vi "Create MCP SSE Response.vi"(8 "error in (no error)":errorcluster) -> (0 "error out":errorcluster, 1 "cancelled":refnum<queue>, 2 "events":refnum<queue>, 3 "MCP SSE Response out":refnum<class "MCP SSE Response.lvclass">)   [LabVIEW 2020, in "MCP Server.lvlib" / "MCP SSE Response.lvclass"]
doc: "Creates an MCP SSE Response ready to be returned from an IG HTTP Server request handler. Obtains the events queue (string; one complete, formatted SSE event per element, an empty string ends the stream) and the cancelled flag (a single-element Boolean queue, initialised to FALSE and set to TRUE by Abort Stream), stores both in the object, and sets status 200 and the headers Content-Type: text/event-stream, Cache-Control: no-cache, X-Accel-Buffering: no and Transfer-Encoding: chunked. The IG HTTP Server frames a response of unknown length in chunks but does not add that header itself; without it a client reads the chunk sizes as part of the body. The caller owns both queues and must release them when the stream is finished."
uses:
  MCP SSE Response.lvclass
  C:/Program Files/National Instruments/LabVIEW 2026/vi.lib/IlluminatedG/IG HTTP Utils/HTTP Utils/Response/Response.lvclass
  MCP SSE Response.lvclass/MCP SSE Response.ctl
  <vilib>/IlluminatedG/IG HTTP Utils/HTTP Utils/Response/Response.lvclass
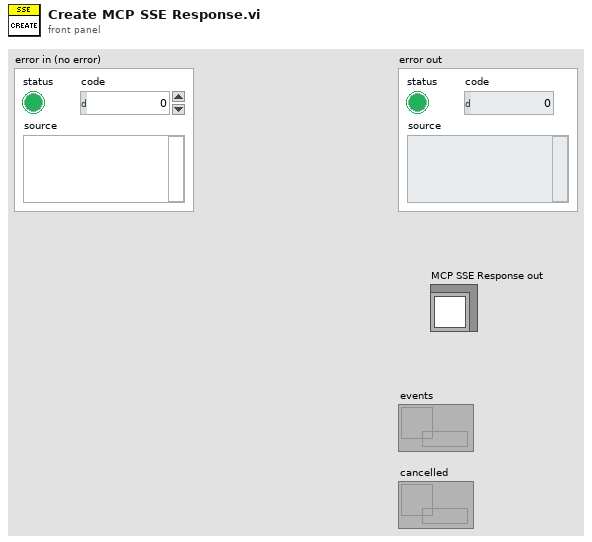
[diagram p1: front panel]
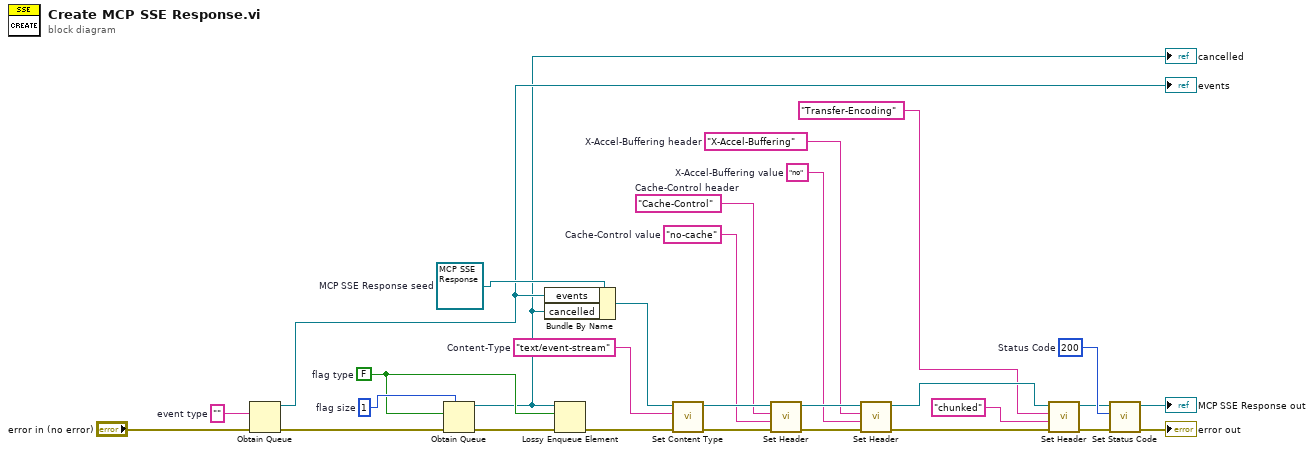
[diagram p0: block diagram]
diagram:
  w11 = u16 200  # Status Code
  w12 = "no"  # X-Accel-Buffering value
  w13 = "X-Accel-Buffering"  # X-Accel-Buffering header
  w16 = "no-cache"  # Cache-Control value
  w17 = "Cache-Control"  # Cache-Control header
  w20 = "text/event-stream"  # Content-Type
  w26 = 1  # flag size
  w25 = FALSE  # flag type
  w29 = ""  # event type
  w23 = refnum<class "MCP SSE Response.lvclass"> refnum  # MCP SSE Response seed
  n1 = Obtain Queue(element data type=w29, error in (no error)="error in (no error)") -> (queue out=w8:refnum<queue>, error out=w27:errorcluster)  [unwired: 3 in, 1 out]
  "events" <- w8
  n2 = Obtain Queue(max queue size (-1, unlimited)=w26, element data type=w25, error in (no error)=w27) -> (queue out=w7:refnum<queue>, error out=w24:errorcluster)  [unwired: 2 in, 1 out]
  "cancelled" <- w7
  n3 = Bundle By Name(cluster=w23, "events"=w8, "cancelled"=w7) -> (w21:refnum<class "MCP SSE Response.lvclass">)
  n4 = Lossy Enqueue Element(queue=w7, element=w25, error in (no error)=w24) -> (error out=w22:errorcluster)  [unwired: 3 out]
  n5 = call <vilib>:"Set Content Type.vi"("error in (no error)"=w22, "Content-Type"=w20, "Response in"=w21) -> ("error out"=w19:errorcluster, "Response out"=w18:refnum<class "MCP SSE Response.lvclass">)  [unwired: 7 in]
  n6 = call <vilib>:"Set Header.vi"("error in (no error)"=w19, "Value"=w16, "Header"=w17, "Response in"=w18) -> ("error out"=w15:errorcluster, "Response out"=w14:refnum<class "MCP SSE Response.lvclass">)  [unwired: 5 in, 1 out]
  n7 = call <vilib>:"Set Header.vi"("error in (no error)"=w15, "Value"=w12, "Header"=w13, "Response in"=w14) -> ("error out"=w3:errorcluster, "Response out"=w4:refnum<class "MCP SSE Response.lvclass">)  [unwired: 5 in, 1 out]
  n8 = call <vilib>:"Set Header.vi"("error in (no error)"=w3, "Value"="chunked", "Header"="Transfer-Encoding", "Response in"=w4) -> ("error out"=w5:errorcluster, "Response out"=w6:refnum<class "MCP SSE Response.lvclass">)  [unwired: 5 in, 1 out]
  n9 = call <vilib>:"Set Status Code.vi"("error in (no error)"=w5, "Status Code"=w11, "Response in"=w6) -> ("error out"=→"error out":errorcluster, "Response out"=→"MCP SSE Response out":refnum<class "MCP SSE Response.lvclass">)  [unwired: 7 in]
